vi "Ecrire config KELLER.vi"(2 "error in (no error)":errorcluster caption="entrée d'erreur (pas d'erreur)", 3 "refnum":T1) -> (0 "error out":errorcluster, 1 "refnum out":T1)   [LabVIEW 2022 SP3]
uses:
  <vilib>/Utility/config.llb/Config Data RefNum.ctl
  Variables globales/Variable glob Keller.vi
  <vilib>/Utility/config.llb/Write Key (String).vi
  <vilib>/Utility/config.llb/Write Key (Boolean).vi
  <vilib>/Utility/config.llb/NI_LVConfig.lvlib
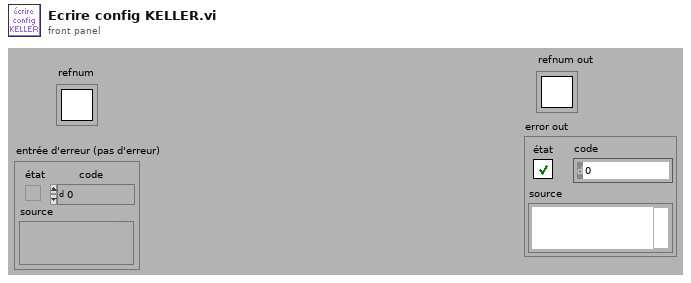
[diagram p1: front panel]
types:
  T1 = typedef "NI_LVConfig.lvlib/Config Data RefNum.ctl" = refnum<k1>
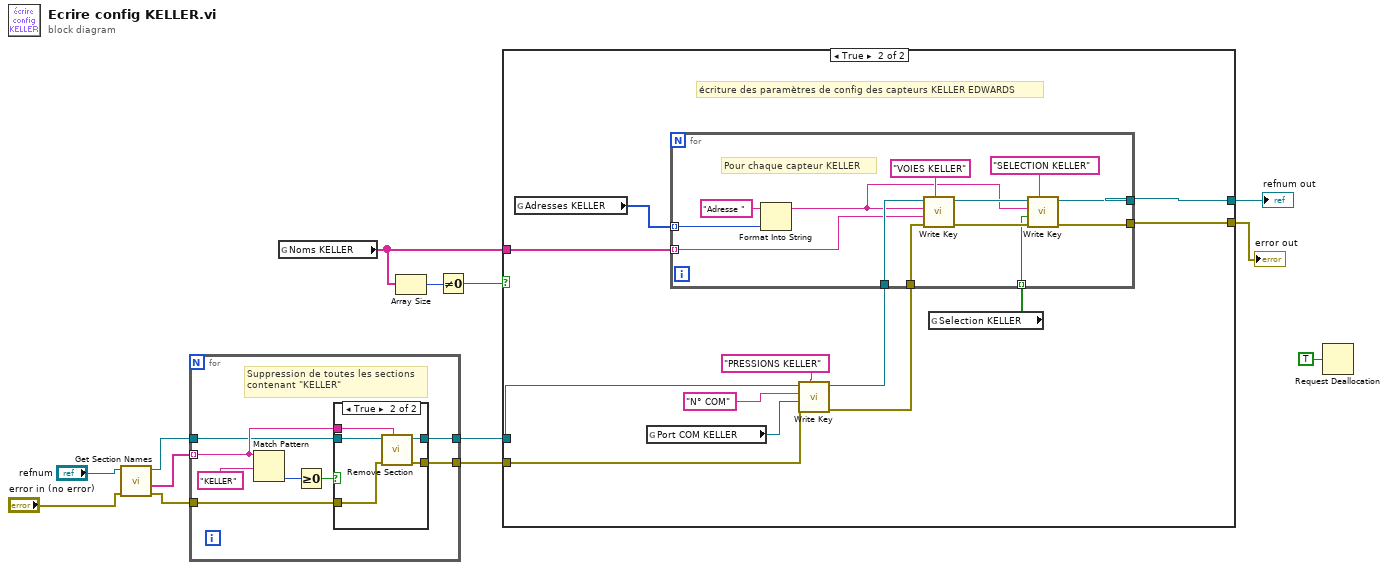
[diagram p0: block diagram]
diagram:
  n1 = call <vilib>:"Get Section Names.vi"("error in (no error)"="error in (no error)", "refnum"="refnum") -> ("error out"=w11:errorcluster, "section names"=w13:string[], "refnum out"=w12:T1)  [unwired: 7 in]
  n2 = for {
    tunnel: w13 -> [w18] mode=indexing
    tunnel: w12 -> [w17]
    tunnel: w11 -> [w16]
    tunnel: [w15] -> w8
    tunnel: [w14] -> w7
    # "Suppression de toutes les sections\ncontenant \"KELLER\""
    n3 = Match Pattern(string=w18, regular expression="KELLER" ("expression régulière")) -> (offset past match=w20:i32)  [unwired: 1 in, 3 out]
    n4 = Greater Or Equal To 0?(x=w20) -> (x >= 0?=w19:bool)
    n5 = case shown="True" w19 {
      tunnel: w18 -> [_ w28]
      tunnel: w17 -> [w23 w27]
      tunnel: w16 -> [w22 w26]
      tunnel: [w23 w25] -> w15
      tunnel: [w22 w24] -> w14
      frame False {
      }
      frame True {
        n6 = call <vilib>:"Remove Section.vi"("section"=w28, "error in (no error)"=w26, "refnum"=w27) -> ("error out"=w24:errorcluster, "refnum out"=w25:T1)  [unwired: 6 in, 1 out]
      }
    }
  }
  n7 = global read "Variable glob Keller.vi" "Noms KELLER"() -> (w6:string[])
  n8 = Array Size(array=w6) -> (size(s)=w5:i32)
  n9 = Not Equal To 0?(x=w5) -> (x != 0?=w4:bool)
  n10 = case shown="True" w4 {
    tunnel: w8 -> [w30 w42]
    tunnel: w7 -> [w29 w41]
    tunnel: w6 -> [_ w36]
    tunnel: [w30 w32] -> w3
    tunnel: [w29 w31] -> w2
    frame False {
    }
    frame True {
      # "écriture des paramètres de config des capteurs KELLER EDWARDS"
      n11 = global read "Variable glob Keller.vi" "Adresses KELLER"() -> (w38:i16[])
      n12 = global read "Variable glob Keller.vi" "Port COM KELLER"() -> (w33:refnum<visa-resource-name>)
      n13 = call-poly <vilib>:"Write Key.vi"("section"="PRESSIONS KELLER", "error in (no error)"=w41, "value"=w33, "key"="N° COM", "refnum"=w42) -> ("error out"=w40:errorcluster, "refnum out"=w39:T1)  [unwired: 4 in, 1 out]
      n14 = global read "Variable glob Keller.vi" "Selection KELLER"() -> (w37:bool[])
      n15 = for {
        tunnel: w39 -> [w55]
        tunnel: w40 -> [w54]
        tunnel: [w46] -> w31
        tunnel: [w47] -> w32
        tunnel: w36 -> [w52] mode=indexing
        tunnel: w38 -> [w51] mode=indexing
        tunnel: w37 -> [w43] mode=indexing
        # "Pour chaque capteur KELLER"
        n16 = Format Into String(initial string="Adresse " ("chaîne initiale"), w51) -> (resulting string=w44:string)  [unwired: 2 in, 1 out]
        n17 = call-poly <vilib>:"Write Key.vi"("section"="VOIES KELLER", "error in (no error)"=w54, "value"=w52, "key"=w44, "refnum"=w55) -> ("error out"=w48:errorcluster, "refnum out"=w49:T1)  [unwired: 4 in, 1 out]
        n18 = call-poly <vilib>:"Write Key.vi"("section"="SELECTION KELLER", "error in (no error)"=w48, "value"=w43, "key"=w44, "refnum"=w49) -> ("error out"=w46:errorcluster, "refnum out"=w47:T1)  [unwired: 4 in, 1 out]
      }
    }
  }
  "refnum out" <- w3
  "error out" <- w2
  n19 = Request Deallocation(TRUE ("flag")) -> ()
